vi "odczyt4.vi"(8 "error in":errorcluster, 11 "Path":path) -> (0 "error out":errorcluster, 3 "Raw Data":T1)   [LabVIEW 2025]
uses:
  Lab 3/Control Raw.ctl
panel:
  out "BPM":i32[](array[numeric])
  out "Time":timestamp[](array[timestamp])
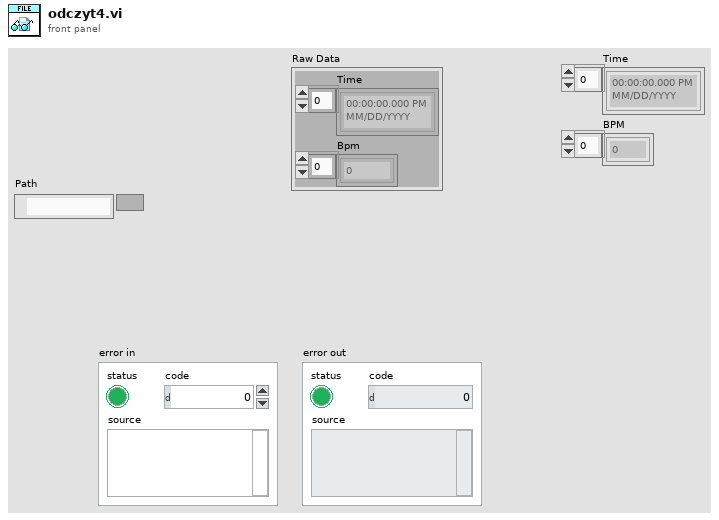
[diagram p1: front panel]
types:
  T1 = typedef "Control Raw.ctl" = cluster{"Time":timestamp[], "Bpm":i32[]}
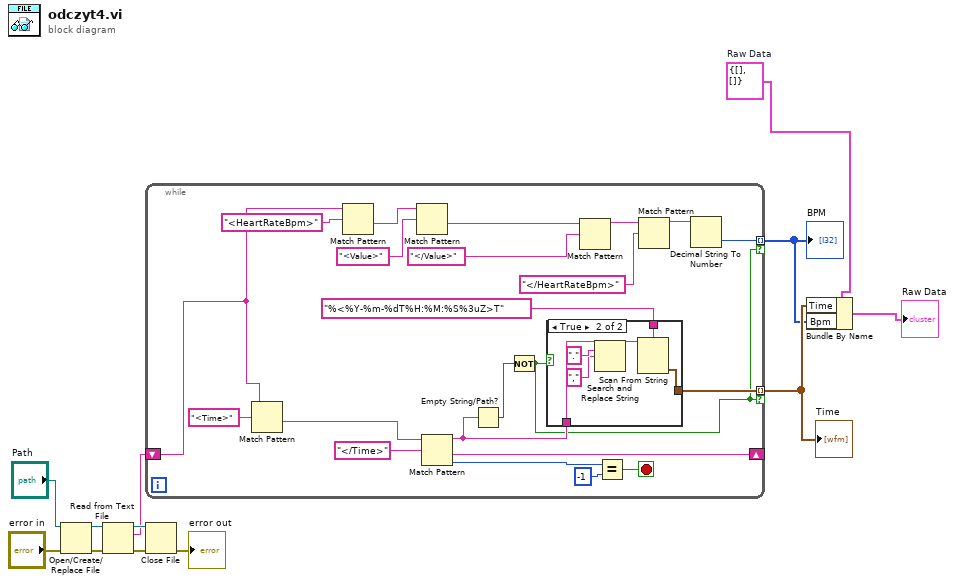
[diagram p0: block diagram]
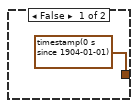
[diagram p2: hidden frame]
diagram:
  w2 = T1 {"Time"=[], "Bpm"=[]}  # Raw Data
  n1 = Open/Create/Replace File(file path (use dialog)="Path", error in="error in") -> (refnum out=w11:refnum<file>, error out=w8:errorcluster)  [unwired: 4 in, 1 out]
  n2 = Read from Text File(file (use dialog)=w11, error in=w8) -> (refnum out=w10:refnum<file>, text=w5:string, error out=w7:errorcluster)  [unwired: 2 in, 1 out]
  n3 = while {
    tunnel: [w32] -> w3 mode=indexing if=w13
    tunnel: [w31] -> w4 mode=indexing if=w13
    shift-right: [w28] -> _
    shift-left: w5 -> [w24]
    stop <- w29 stop-if-true
    n4 = Match Pattern(string=w24, regular expression="<Time>") -> (after substring=w26:string)  [unwired: 1 in, 3 out]
    n5 = Match Pattern(string=w24, regular expression="<HeartRateBpm>") -> (after substring=w21:string)  [unwired: 1 in, 3 out]
    n6 = Match Pattern(string=w21, regular expression="<Value>") -> (after substring=w20:string)  [unwired: 1 in, 3 out]
    n7 = Match Pattern(string=w26, regular expression="</Time>") -> (before substring=w15:string, after substring=w28:string, offset past match=w16:i32)  [unwired: 1 in, 1 out]
    n8 = Empty String/Path?(string/path=w15) -> (empty?=w14:bool)
    n9 = Not(x=w14) -> (.not. x?=w13:bool)
    n10 = case shown="True" w13 {
      tunnel: "%<%Y-%m-%dT%H:%M:%S%3uZ>T" -> [_ w41]
      tunnel: [timestamp(0 s since 1904-01-01) w40] -> w31
      tunnel: w15 -> [_ w36]
      frame False {
      }
      frame True {
        n11 = Search and Replace String(input string=w36, search string=".", replace string="," ("replace string (\"\")")) -> (result string=w37:string)  [unwired: 5 in, 3 out]
        n12 = Scan From String(format string=w41, input string=w37) -> (output 1=w40:timestamp)  [unwired: 3 in, 3 out]
      }
    }
    n13 = Match Pattern(string=w20, regular expression="</Value>") -> (before substring=w19:string)  [unwired: 1 in, 3 out]
    n14 = Equal?(x=w16, y=-1) -> (x = y?=w29:bool)
    n15 = Match Pattern(string=w19, regular expression="</HeartRateBpm>") -> (before substring=w33:string)  [unwired: 1 in, 3 out]
    n16 = Decimal String To Number(string=w33) -> (number=w32:i32)  [unwired: 2 in, 1 out]
  }
  "Time" <- w4
  "BPM" <- w3
  n17 = Close File(refnum=w10, error in=w7) -> (error out=→"error out":errorcluster)  [unwired: 1 out]
  n18 = Bundle By Name(cluster=w2, "Time"=w4, "Bpm"=w3) -> (→"Raw Data":T1)
